vi "Print Diagram Frames.vi"(11 "Command Line Arguments":string[](array[string])) -> (2 "Output":string, 3 "Exit Code":i32)   [LabVIEW 2020]
doc: "Prints the block diagram of one VI to HTML and PNG with every case frame, and writes a text file that says which structure and frame each picture shows. CI helper driven by tools\\ci\\New-ViDiffReport.ps1 through LabVIEW CLI RunVI (LabVIEWCLI -OperationName RunVI -VIPath this VI arg0 arg1 arg2).\n\nCommand Line Arguments: [0] absolute path of the VI to print, [1] absolute path of the HTML file to write (its folder is also the image directory and is created if missing), [2] absolute path of the frame list text file (its folder is created if missing).\n\nPrint.VI To HTML runs with Format Complete. LabVIEW writes base d.png for the whole diagram with the visible frames and base d1.png .. dN.png for the hidden frames.\n\nThe frame list has one line per frame of every multi-frame structure (Case, Event, Stacked Sequence, Disable structures), nested ones included, tab separated: structure number (1-based, in print order), class name, label text, frame index, 1 if visible frame else 0, frame name (case structures only, surrounding blanks trimmed). Lines end in LF. The lines follow LabVIEW's own print order, so the lines with visible flag 0 are the pictures d1..dN in that order. Measured rule: on each diagram the structures are visited in REVERSE order of All Objects[], each structure's frames in index order, and each frame is immediately followed by the structures nested in it (pre-order). Loops and other single-diagram structures are walked through transparently.\n\nExit Code is 0 on success and 1 on any error, including fewer than three arguments. Output is a one-line summary on success and the error code and source on error."
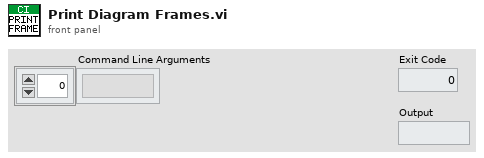
[diagram p1: front panel]
types:
  T1 = enum16{"Custom", "Standard", "Using Panel", "Using SubVI", "Complete"}
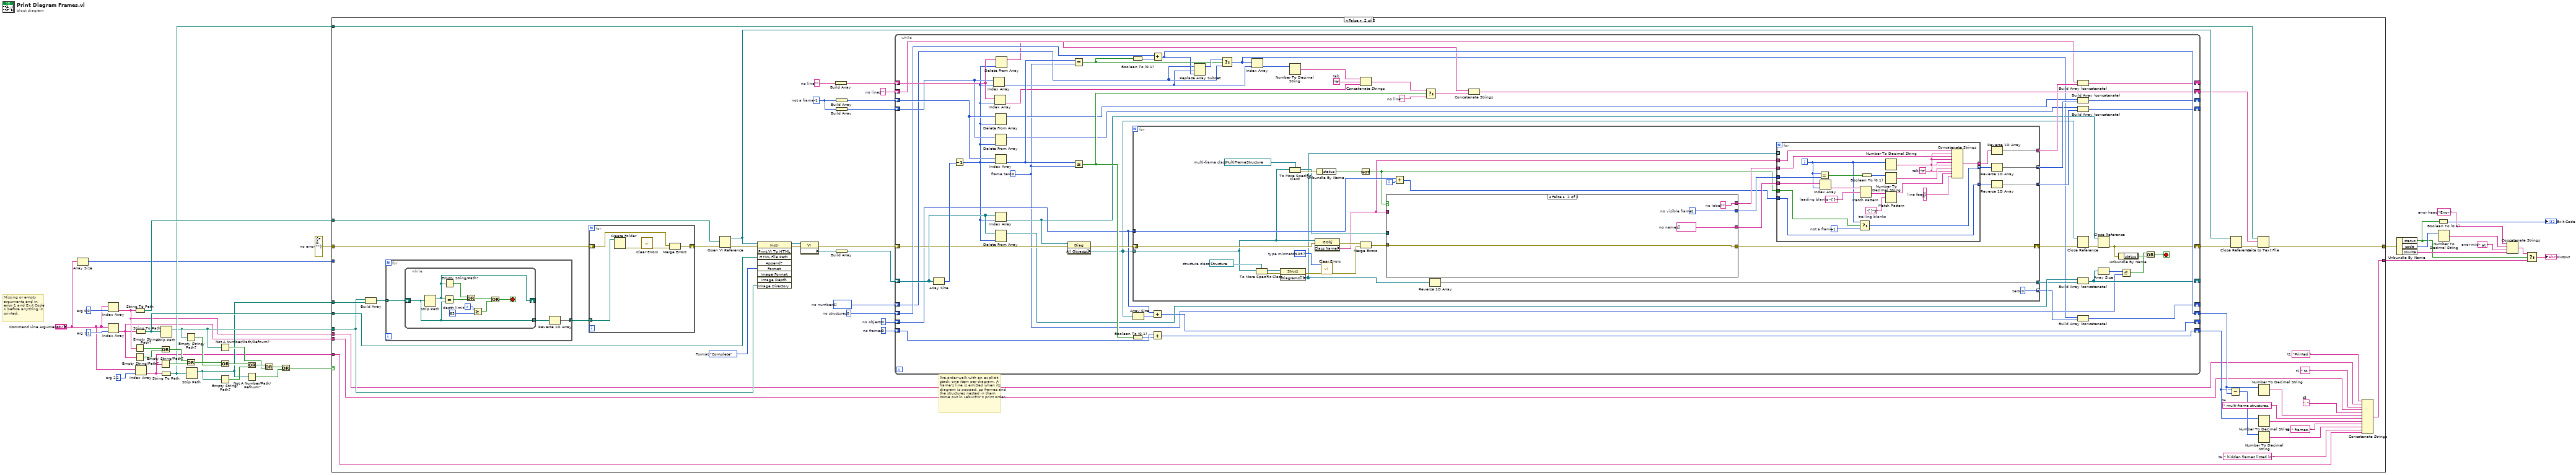
[diagram p0: block diagram]
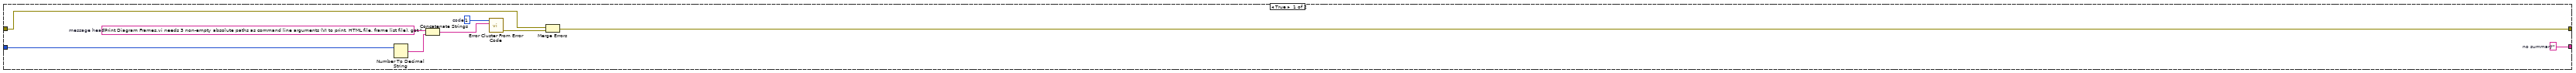
[diagram p2: hidden frame]
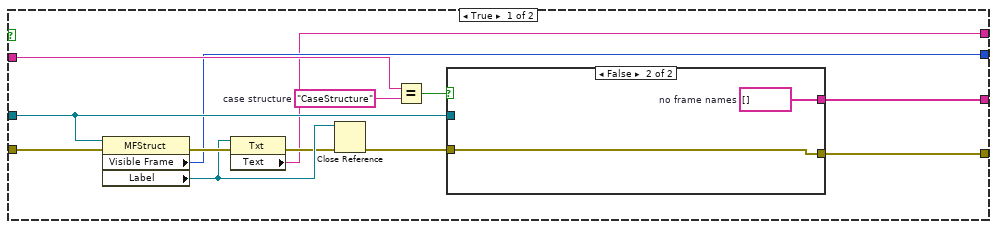
[diagram p3: hidden frame]
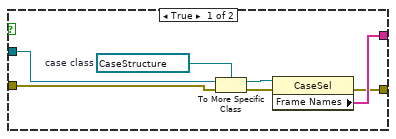
[diagram p4: hidden frame]
diagram:
  w7 = " at "  # error mid
  w9 = "Error "  # error head
  w35 = 2  # arg 2
  w37 = 1  # arg 1
  w38 = 0  # arg 0
  w22 = errorcluster {"status"=FALSE, "code"=0, "source"=""}  # no error
  # "Missing or empty arguments end in error 1 and Exit Code 1 before anything is printed."
  n1 = Array Size(array="Command Line Arguments") -> (size(s)=w16:i32)
  n2 = Index Array(array="Command Line Arguments", index=w38) -> (element=w15:string)
  n3 = Index Array(array="Command Line Arguments", index=w37) -> (element=w14:string)
  n4 = Empty String/Path?(string/path=w15) -> (empty?=w34:bool)
  n5 = Empty String/Path?(string/path=w14) -> (empty?=w33:bool)
  n6 = String To Path(string=w15) -> (path=w21:path)
  n7 = String To Path(string=w14) -> (path=w20:path)
  n8 = Index Array(array="Command Line Arguments", index=w35) -> (element=w13:string)
  n9 = Or(x=w34, y=w33) -> (x .or. y?=w32:bool)
  n10 = Empty String/Path?(string/path=w13) -> (empty?=w31:bool)
  n11 = Strip Path(path=w20) -> (stripped path=w18:path)  [unwired: 1 out]
  n12 = String To Path(string=w13) -> (path=w19:path)
  n13 = Empty String/Path?(string/path=w18) -> (empty?=w29:bool)
  n14 = Or(x=w32, y=w31) -> (x .or. y?=w30:bool)
  n15 = Strip Path(path=w19) -> (stripped path=w17:path)  [unwired: 1 out]
  n16 = Not A Number/Path/Refnum?(number/path/refnum=w18) -> (NaN/Path/Refnum?=w25:bool)
  n17 = Or(x=w30, y=w29) -> (x .or. y?=w28:bool)
  n18 = Empty String/Path?(string/path=w17) -> (empty?=w27:bool)
  n19 = Or(x=w28, y=w27) -> (x .or. y?=w26:bool)
  n20 = Not A Number/Path/Refnum?(number/path/refnum=w17) -> (NaN/Path/Refnum?=w23:bool)
  n21 = Or(x=w26, y=w25) -> (x .or. y?=w24:bool)
  n22 = Or(x=w24, y=w23) -> (x .or. y?=w12:bool)
  n23 = case shown="False" w12 {
    tunnel: w22 -> [w42 w91]
    tunnel: w21 -> [_ w90]
    tunnel: w20 -> [_ w87]
    tunnel: w19 -> [_ w67]
    tunnel: w18 -> [_ w85]
    tunnel: w17 -> [_ w94]
    tunnel: w16 -> [w47 _]
    tunnel: w15 -> [_ w60]
    tunnel: w14 -> [_ w58]
    tunnel: w13 -> [_ w50]
    tunnel: [w40 w49] -> w3
    tunnel: [w39 w48] -> w11
    frame True {
      w40 = ""  # no summary
      w44 = 1  # code
      w46 = "Print Diagram Frames.vi needs 3 non-empty absolute paths as command line arguments (VI to print, HTML file, frame list file), got "  # message head
      n24 = Number To Decimal String(number=w47) -> (decimal integer string=w45:string)  [unwired: 1 in]
      n25 = Concatenate Strings(w46, w45) -> (w43:string)
      n26 = call <vilib>:"Error Cluster From Error Code.vi"("error message (\"\")"=w43, "error code (0)"=w44) -> ("error out"=w41:errorcluster)  [unwired: 7 in]
      n27 = Merge Errors(w42, w41) -> (w39:errorcluster)
    }
    frame False {
      w51 = " hidden frames listed in "  # t6
      w53 = " frames, "  # t5
      w55 = " multi-frame structures, "  # t4
      w57 = ": "  # t3
      w59 = " to "  # t2
      w61 = "Printed "  # t1
      w74 = 0  # no objects
      w71 = 0  # no frames
      w72 = 0  # no structures
      w73 = ""  # no lines
      w75 = i32[] []  # no numbers
      w80 = -1  # not a frame
      w81 = ""  # no line
      w86 = T1."Complete"  # Format
      # "Pre-order walk with an explicit stack: one item per diagram. A frame's line is emitted when its diagram is popped, so frames and the structures nested in them come out in LabVIEW's print order."
      n28 = Build Array(w85, w94) -> (w93:path[])
      n29 = for {
        tunnel: w93 -> [w238] mode=indexing
        tunnel: [w236] -> w92 mode=concatenating
        n30 = while {
          shift-right: [w247] -> _
          shift-left: w238 -> [w240]
          tunnel: [w240] -> w237 mode=indexing
          i -> [w239]
          stop <- w241 stop-if-true
          w246 = 63  # depth limit
          n31 = Strip Path(path=w240) -> (stripped path=w247:path)  [unwired: 1 out]
          n32 = Equal?(x=w247, y=w240) -> (x = y?=w244:bool)
          n33 = Empty String/Path?(string/path=w247) -> (empty?=w245:bool)
          n34 = Or(x=w245, y=w244) -> (x .or. y?=w243:bool)
          n35 = Greater Or Equal?(x=w239, y=w246) -> (x >= y?=w242:bool)
          n36 = Or(x=w243, y=w242) -> (x .or. y?=w241:bool)
        }
        n37 = Reverse 1D Array(array=w237) -> (reversed array=w236:path[])
      }
      n38 = for {
        tunnel: w92 -> [w235] mode=indexing
        shift-right: [w231] -> w89
        shift-left: w91 -> [w233]
        n39 = Create Folder(path (use dialog)=w235) -> (error out=w234:errorcluster)  [unwired: 2 in, 2 out]
        n40 = call <vilib>:"Clear Errors.vi"("error in (no error)"=w234) -> ("error out"=w232:errorcluster)  [unwired: 5 in, 1 out]
        n41 = Merge Errors(w233, w232) -> (w231:errorcluster)
      }
      n42 = Open VI Reference(vi path=w90, error in (no error)=w89) -> (vi reference=w69:refnum<vi>, error out=w88:errorcluster)  [unwired: 4 in]
      n43 = invoke class="Instr" method="Print.VI To HTML"(reference=w69, error in=w88, "HTML File Path"=w87, "Format"=w86, "Image Directory"=w85) -> (reference out=w84:refnum<vi>, error out=w83:errorcluster)  [unwired: 4 in, 7 out]
      n44 = property class="VI"(reference=w84, error in=w83) -> (error out=w70:errorcluster, "Block Diagram"=w82:refnum<vi>)  [unwired: 1 out]
      n45 = Build Array(w81) -> (w78:string[])
      n46 = Build Array(w80) -> (w77:i32[])
      n47 = Build Array(w80) -> (w76:i32[])
      n48 = Build Array(w82) -> (w79:refnum<vi>[])
      n49 = while {
        shift-right: [w101] -> _
        shift-left: w79 -> [w150]
        shift-right: [w118] -> _
        shift-left: w78 -> [w149]
        shift-right: [w115] -> _
        shift-left: w77 -> [w148]
        shift-right: [w112] -> _
        shift-left: w76 -> [w147]
        shift-right: [w109] -> _
        shift-left: w75 -> [w136]
        shift-right: [w106] -> _
        shift-left: w74 -> [w108]
        shift-right: [w125] -> w66
        shift-left: w73 -> [w127]
        shift-right: [w139] -> w64
        shift-left: w72 -> [w144]
        shift-right: [w140] -> w63
        shift-left: w71 -> [w142]
        shift-right: [w98] -> w68
        shift-left: w70 -> [w124]
        stop <- w95 stop-if-true
        w128 = ""  # no line
        w132 = "\t"  # tab
        w99 = 0  # frame zero
        n50 = Array Size(array=w150) -> (size(s)=w151:i32)
        n51 = Decrement(x=w151) -> (x-1=w146:i32)
        n52 = Index Array(array=w147, index=w146) -> (element=w135:i32)
        n53 = Index Array(array=w149, index=w146) -> (element=w131:string)
        n54 = Delete From Array(array=w148, index=w146) -> (array with subset deleted=w117:i32[])  [unwired: 1 in, 1 out]
        n55 = Delete From Array(array=w147, index=w146) -> (array with subset deleted=w114:i32[])  [unwired: 1 in, 1 out]
        n56 = Index Array(array=w148, index=w146) -> (element=w145:i32)
        n57 = Index Array(array=w150, index=w146) -> (element=w103:refnum<vi>)
        n58 = Delete From Array(array=w150, index=w146) -> (array with subset deleted=w122:refnum<vi>[])  [unwired: 1 in, 1 out]
        n59 = Delete From Array(array=w149, index=w146) -> (array with subset deleted=w120:string[])  [unwired: 1 in, 1 out]
        n60 = property class="Diag"(reference=w103, error in=w124) -> (error out=w123:errorcluster, "All Objects[]"=w105:refnum<vi>[])  [unwired: 1 out]
        n61 = Equal?(x=w145, y=w99) -> (x = y?=w137:bool)
        n62 = Greater Or Equal?(x=w145, y=w99) -> (x >= y?=w129:bool)
        n63 = Boolean To (0,1)(Boolean=w137) -> (0, 1=w143:i16)
        n64 = Boolean To (0,1)(Boolean=w129) -> (0, 1=w141:i16)
        n65 = for {
          tunnel: w105 -> [w174] mode=indexing
          tunnel: w108 -> [w183]
          shift-right: [w168] -> w104
          shift-left: w123 -> [w182]
          tunnel: [w157] -> w121 mode=concatenating
          tunnel: [w156] -> w119 mode=concatenating
          tunnel: [w155] -> w116 mode=concatenating
          tunnel: [w154] -> w113 mode=concatenating
          tunnel: [w153] -> w110 mode=indexing
          i -> [w152]
          w153 = 0  # zero
          w178 = 1057  # type mismatch
          w173 = refnum<vi> refnum  # multi-frame class
          w181 = refnum<vi> refnum  # structure class
          n66 = To More Specific Class(target class=w181, reference=w174) -> (specific class reference=w180:refnum<vi>, error out=w179:errorcluster)  [unwired: 1 in]
          n67 = property class="Struct"(reference=w180, error in=w179) -> (error out=w177:errorcluster, "Diagrams[]"=w161:refnum<vi>[])  [unwired: 1 out]
          n68 = To More Specific Class(target class=w173, reference=w174) -> (specific class reference=w170:refnum<vi>, error out=w172:errorcluster)  [unwired: 1 in]
          n69 = property class="GObj"(reference=w174, error in=w182) -> (error out=w176:errorcluster, "Class Name"=w165:string)  [unwired: 1 out]
          n70 = Unbundle By Name(w172) -> ("status"=w171:bool)
          n71 = call <vilib>:"Clear Errors.vi"("error in (no error)"=w177, "specific error code to clear (0: all)"=w178) -> ("error out"=w175:errorcluster)  [unwired: 4 in, 1 out]
          n72 = Not(x=w171) -> (.not. x?=w163:bool)
          n73 = Merge Errors(w176, w175) -> (w169:errorcluster)
          n74 = case shown="False" w163 {
            tunnel: w170 -> [w211 _]
            tunnel: w169 -> [w217 w227]
            tunnel: w165 -> [w213 _]
            tunnel: [w208 w230] -> w166
            tunnel: [w207 w229] -> w164
            tunnel: [w206 w228] -> w167
            tunnel: [w205 w227] -> w168
            frame True {
              w212 = "CaseStructure"  # case structure
              n75 = property class="MFStruct"(reference=w211, error in=w217) -> (error out=w216:errorcluster, "Visible Frame"=w208:u32, "Label"=w215:refnum<vi>)  [unwired: 1 out]
              n76 = property class="Txt"(reference=w215, error in=w216) -> (error out=w214:errorcluster, "Text"=w207:string)  [unwired: 1 out]
              n77 = Close Reference(reference=w215, error in (no error)=w214) -> (error out=w210:errorcluster)
              n78 = Equal?(x=w213, y=w212) -> (x = y?=w209:bool)
              n79 = case shown="False" w209 {
                tunnel: w211 -> [w224 _]
                tunnel: w210 -> [w223 w225]
                tunnel: [w219 w226] -> w206
                tunnel: [w218 w225] -> w205
                frame True {
                  w222 = refnum<vi> refnum  # case class
                  n80 = To More Specific Class(target class=w222, reference=w224, error in=w223) -> (specific class reference=w221:refnum<vi>, error out=w220:errorcluster)
                  n81 = property class="CaseSel"(reference=w221, error in=w220) -> (error out=w218:errorcluster, "Frame Names"=w219:string[])  [unwired: 1 out]
                }
                frame False {
                  w226 = string[] []  # no frame names
                }
              }
            }
            frame False {
              w228 = string[] []  # no names
              w229 = ""  # no label
              w230 = -1  # no visible frame
            }
          }
          n82 = Add(x=w183, y=w152) -> (x+y=w162:i32)
          n83 = Reverse 1D Array(array=w161) -> (reversed array=w157:refnum<vi>[])
          n84 = for {
            tunnel: w161 -> [_] mode=indexing
            tunnel: w167 -> [w204]
            tunnel: w166 -> [w199]
            tunnel: w165 -> [w196]
            tunnel: w164 -> [w195]
            tunnel: w163 -> [w189]
            tunnel: w162 -> [w185]
            tunnel: [w187] -> w160 mode=indexing
            tunnel: [w186] -> w159 mode=indexing
            tunnel: [w185] -> w158 mode=indexing
            i -> [w184]
            w188 = -1  # not a frame
            w190 = "\n"  # line feed
            w192 = "\t"  # tab
            w200 = "[ ]*$"  # trailing blanks
            w202 = "^[ ]*"  # leading blanks
            n85 = Equal?(x=w184, y=w199) -> (x = y?=w198:bool)
            n86 = Index Array(array=w204, index=w184) -> (element=w203:string)
            n87 = Select(t=w184, s=w189, f=w188) -> (s? t:f=w186:i32)
            n88 = Match Pattern(string=w203, regular expression=w202) -> (after substring=w201:string)  [unwired: 1 in, 3 out]
            n89 = Boolean To (0,1)(Boolean=w198) -> (0, 1=w197:i16)
            n90 = Number To Decimal String(number=w184) -> (decimal integer string=w194:string)  [unwired: 1 in]
            n91 = Number To Decimal String(number=w197) -> (decimal integer string=w193:string)  [unwired: 1 in]
            n92 = Match Pattern(string=w201, regular expression=w200) -> (before substring=w191:string)  [unwired: 1 in, 3 out]
            n93 = Concatenate Strings(w196, w192, w195, w192, w194, w192, w193, w192, w191, w190) -> (w187:string)
          }
          n94 = Reverse 1D Array(array=w160) -> (reversed array=w156:string[])
          n95 = Reverse 1D Array(array=w159) -> (reversed array=w155:i32[])
          n96 = Reverse 1D Array(array=w158) -> (reversed array=w154:i32[])
        }
        n97 = Array Size(array=w105) -> (size(s)=w107:i32)
        n98 = Add(x=w108, y=w107) -> (x+y=w106:i32)
        n99 = Add(x=w142, y=w141) -> (x+y=w140:i32)
        n100 = Add(x=w144, y=w143) -> (x+y=w139:i32)
        n101 = Replace Array Subset(array=w136, new element=w139, index=w135) -> (w138:i32[])
        n102 = Select(t=w138, s=w137, f=w136) -> (s? t:f=w111:i32[])
        n103 = Index Array(array=w111, index=w135) -> (element=w134:i32)
        n104 = Number To Decimal String(number=w134) -> (decimal integer string=w133:string)  [unwired: 1 in]
        n105 = Concatenate Strings(w133, w132, w131) -> (w130:string)
        n106 = Select(t=w130, s=w129, f=w128) -> (s? t:f=w126:string)
        n107 = Concatenate Strings(w127, w126) -> (w125:string)
        n108 = Build Array (concatenate)(w120, w119) -> (w118:string[])
        n109 = Build Array (concatenate)(w117, w116) -> (w115:i32[])
        n110 = Build Array (concatenate)(w114, w113) -> (w112:i32[])
        n111 = Close Reference(reference=w105, error in (no error)=w104) -> (error out=w102:errorcluster)
        n112 = Build Array (concatenate)(w122, w121) -> (w101:refnum<vi>[])
        n113 = Build Array (concatenate)(w111, w110) -> (w109:i32[])
        n114 = Close Reference(reference=w103, error in (no error)=w102) -> (error out=w98:errorcluster)
        n115 = Array Size(array=w101) -> (size(s)=w100:i32)
        n116 = Unbundle By Name(w98) -> ("status"=w96:bool)
        n117 = Less Or Equal?(x=w100, y=w99) -> (x <= y?=w97:bool)
        n118 = Or(x=w97, y=w96) -> (x .or. y?=w95:bool)
      }
      n119 = Subtract(x=w63, y=w64) -> (x-y=w62:i32)
      n120 = Close Reference(reference=w69, error in (no error)=w68) -> (error out=w65:errorcluster)
      n121 = Write to Text File(file (use dialog)=w67, text=w66, error in=w65) -> (error out=w48:errorcluster)  [unwired: 1 in, 2 out]
      n122 = Number To Decimal String(number=w64) -> (decimal integer string=w56:string)  [unwired: 1 in]
      n123 = Number To Decimal String(number=w63) -> (decimal integer string=w54:string)  [unwired: 1 in]
      n124 = Number To Decimal String(number=w62) -> (decimal integer string=w52:string)  [unwired: 1 in]
      n125 = Concatenate Strings(w61, w60, w59, w58, w57, w56, w55, w54, w53, w52, w51, w50) -> (w49:string)
    }
  }
  n126 = Unbundle By Name(w11) -> ("status"=w4:bool, "code"=w10:i32, "source"=w6:string)
  n127 = Boolean To (0,1)(Boolean=w4) -> (0, 1=→"Exit Code":i16)
  n128 = Number To Decimal String(number=w10) -> (decimal integer string=w8:string)  [unwired: 1 in]
  n129 = Concatenate Strings(w9, w8, w7, w6) -> (w5:string)
  n130 = Select(t=w5, s=w4, f=w3) -> (s? t:f=→"Output":string)
